vi "Read Language Selection UTF-16 LE.vi"(8 "error in (no error)":errorcluster, 11 "LanguageSelection file":path) -> (0 "error out":errorcluster, 3 "Language Selection":T1)   [LabVIEW 2019, in "Language Selection.lvlib"]
doc: "Convert translation from JSON format.\n- - -\nCopyright (c) 2026, Merecs Engineering GmbH"
uses:
  Language Selection.lvlib
  TypeDefs/Cluster Language Configuration.ctl
  Cluster Settings Data.ctl
  TypeDefs/Cluster Language.ctl
  TypeDefs/Cluster PropertyTranslation.ctl
  TypeDefs/Enum Property Type.ctl
  7aaee674-9885-4f51-b860-93eee7d62f3f.vi
  private/Hex-String To String.vi
  <vilib>/addons/Tools/Unicode/_subVIs/Convert ASCII to UTF-16LE (Scalar).vi
  <vilib>/addons/Tools/Unicode/_subVIs/Convert UTF-16LE to ASCII (Scalar).vi
  <vilib>/JDP Science/JSONtext/JSON text to Variant.vi
  <vilib>/JDP Science/JSONtext/LVClass Serializer/JSONtext LVClass Serializer.lvclass
  <vilib>/addons/Tools/Unicode/UI Unicode Tools.lvlib
panel:
  # "Connector Pane"
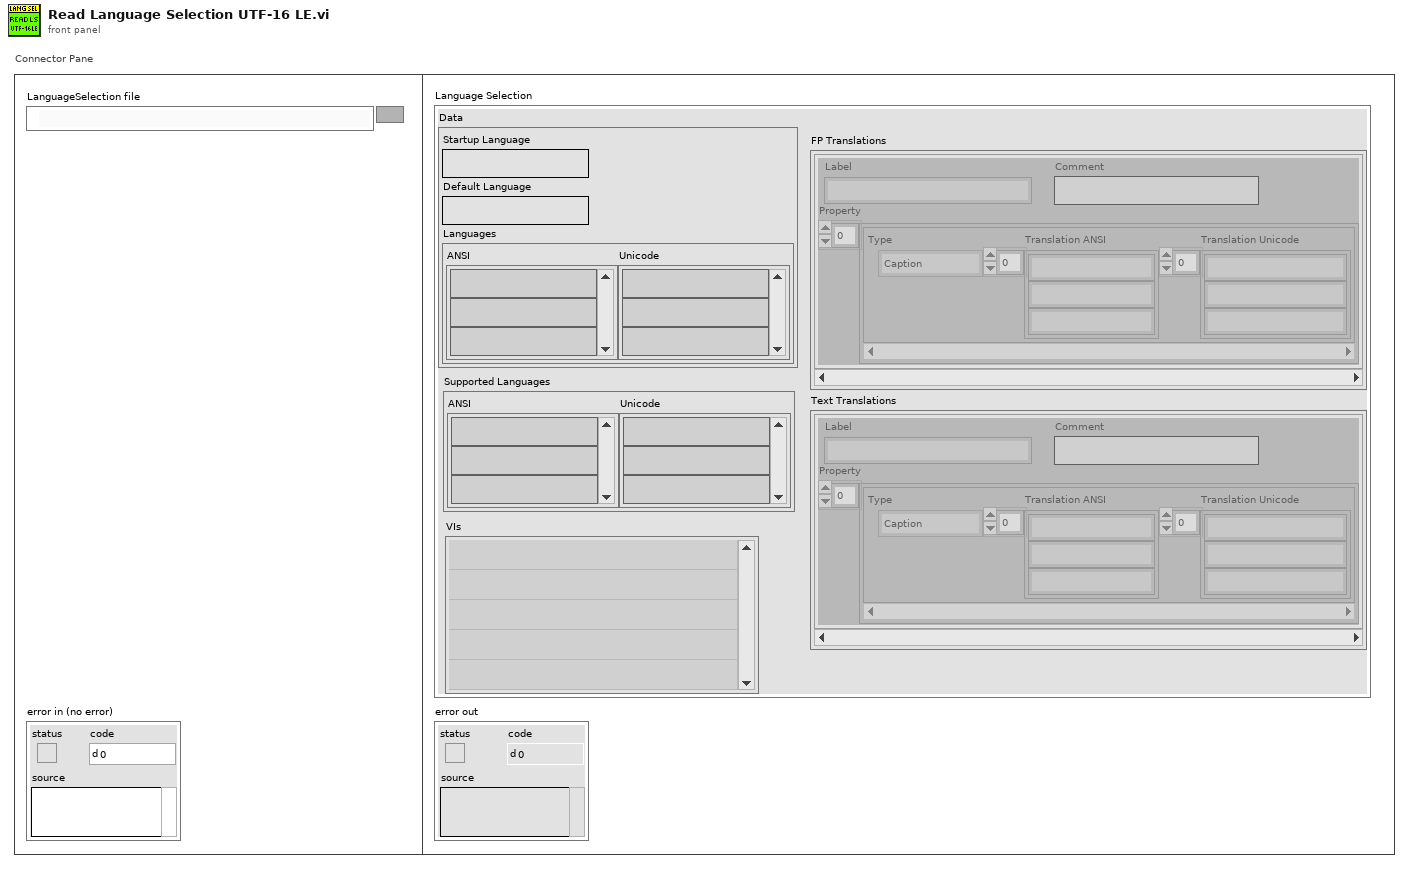
[diagram p1: front panel]
types:
  T1 = typedef "Language Selection.lvlib/Cluster Language Configuration.ctl" = cluster{"Data":T2, "Supported Languages":cluster{"ANSI":string[], "Unicode":string[]}, "VIs":path[], "FP Translations":T3[], "Text Translations":T3[]}
  T2 = typedef "Language Selection.lvlib/Cluster Settings Data.ctl" = cluster{"Startup Language":string, "Default Language":string, "Languages":cluster{"ANSI":string[], "Unicode":string[]}}
  T3 = typedef "Language Selection.lvlib/Cluster Language.ctl" = cluster{"Label":string, "Comment":string, "Property":T4[]}
  T4 = typedef "Language Selection.lvlib/Cluster PropertyTranslation.ctl" = cluster{"Type":T5, "Translation ANSI":string[], "Translation Unicode":string[]}
  T5 = typedef "Language Selection.lvlib/Enum Property Type.ctl" = enum16{"NA", "Caption", "String Value", "Boolean Text", "Ring Strings", "1D Array Elements", "2D Array Elements", "(MC)Listbox Header", "(MC)Listbox Items", "Tab Pages Names", "X & Y GraphChart", "Plot Names", "Table Headers", "Table Items", "TipStrip", "Combobox Strings", "Cursor Name", "Tree Col Headers"}
  T6 = enum16{"open", "replace", "create", "open or create", "replace or create", "replace or create with confirmation"}
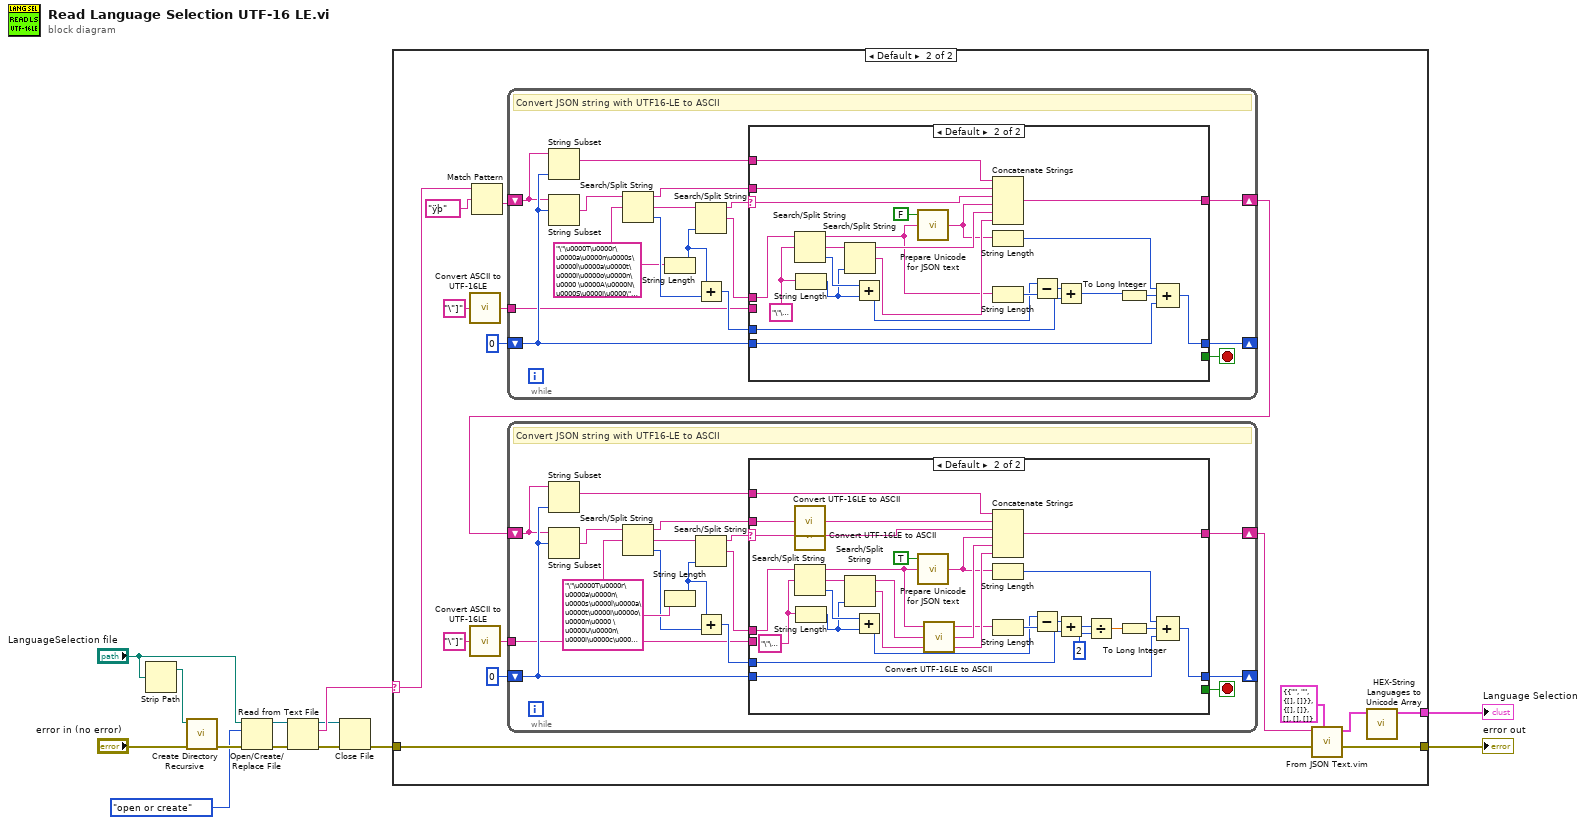
[diagram p0: block diagram]
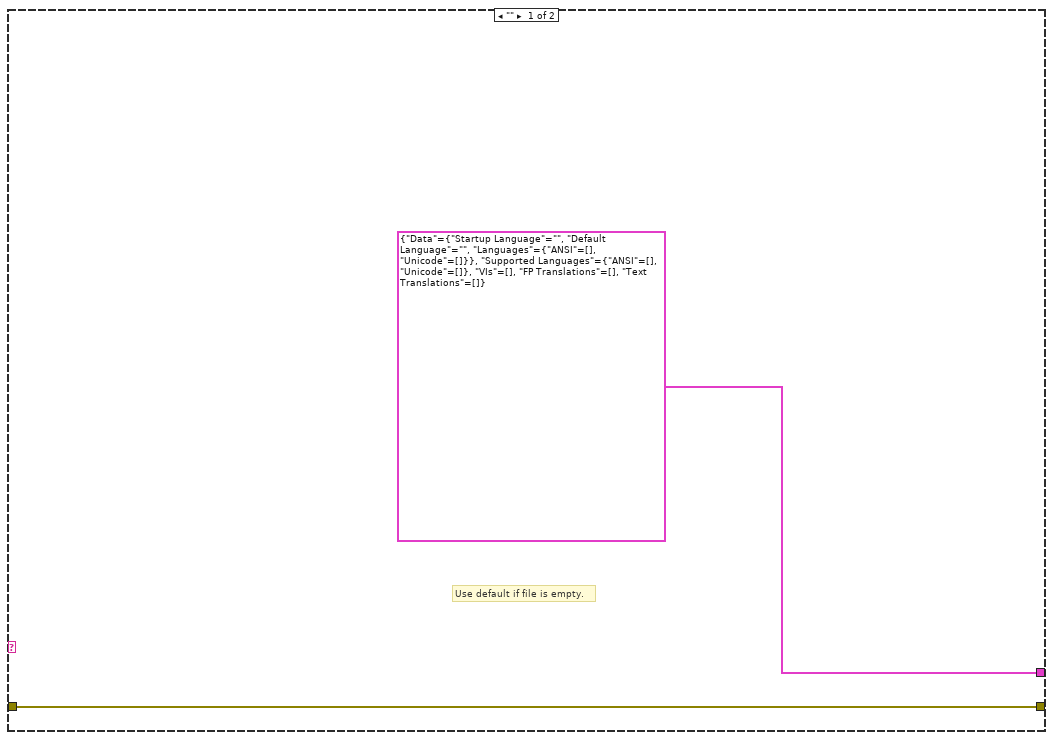
[diagram p2: hidden frame]
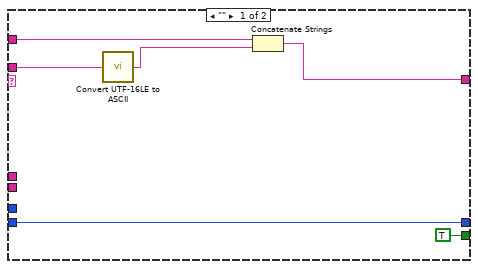
[diagram p3: hidden frame]
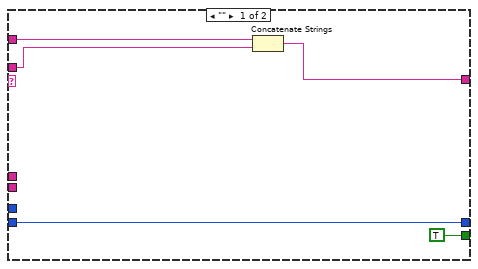
[diagram p4: hidden frame]
diagram:
  n1 = Strip Path(path="LanguageSelection file") -> (stripped path=w9:path)  [unwired: 1 out]
  n2 = call <vilib>:"Create Directory Recursive.vi"("error in (no error)"="error in (no error)", "directory"=w9) -> ("error out"=w7:errorcluster)  [unwired: 3 in, 2 out]
  n3 = Open/Create/Replace File(file path (use dialog)="LanguageSelection file", error in=w7, operation (0:open)=T6."open or create") -> (refnum out=w3:refnum<file>, error out=w4:errorcluster)  [unwired: 3 in, 1 out]
  n4 = Read from Text File(file (use dialog)=w3, error in=w4) -> (refnum out=w1:refnum<file>, text=w10:string, error out=w13:errorcluster)  [unwired: 2 in, 1 out]
  n5 = Close File(refnum=w1, error in=w13) -> (error out=w2:errorcluster)  [unwired: 1 out]
  n6 = case shown="Default" w10 {
    selector: w10 -> [_ w17]
    tunnel: w2 -> [w15 w29]
    tunnel: [w15 w28] -> w12
    tunnel: [T1 {"Data"={"Startup Language"="", "Default Language"="", "Languages"={"ANSI"=[], "Unicode"=[]}}, "Supported Languages"={"ANSI"=[], "Unicode"=[]}, "VIs"=[], "FP Translations"=[], "Text Translations"=[]} ("Config out") w16] -> w11
    frame "" {
      # "Use default if file is empty."
    }
    frame Default {
      n7 = call-poly <vilib>:"Convert ASCII to UTF-16LE.vi"("ASCII"="\"]" ("regular expression")) -> ("Unicode"=w26:string)  [unwired: 4 in]
      n8 = call-poly <vilib>:"Convert ASCII to UTF-16LE.vi"("ASCII"="\"]" ("regular expression")) -> ("Unicode"=w21:string)  [unwired: 4 in]
      n9 = Match Pattern(string=w17, regular expression="ÿþ" ("string")) -> (after substring=w23:string)  [unwired: 1 in, 3 out]
      n10 = while {
        shift-right: [w83] -> w20
        shift-left: w23 -> [w94]
        shift-right: [w96] -> _
        shift-left: 0 -> [w95]
        tunnel: w26 -> [w84]
        stop <- w97 stop-if-true
        w82 = "\"\u0000T\u0000r\u0000a\u0000n\u0000s\u0000l\u0000a\u0000t\u0000i\u0000o\u0000n\u0000 \u0000A\u0000N\u0000S\u0000I\u0000\"\u0000:\u0000[\u0000\"\u0000" ("Unicode 2")
        # "Convert JSON string with UTF16-LE to ASCII"
        n11 = String Subset(string=w94, length (rest)=w95) -> (substring=w93:string)  [unwired: 1 in]
        n12 = String Subset(string=w94, offset (0)=w95) -> (substring=w92:string)  [unwired: 1 in]
        n13 = Search/Split String(string=w92, search string/char (-)=w82) -> (substring before match=w91:string, match + rest of string=w90:string, offset of match=w86:i32)  [unwired: 1 in]
        n14 = String Length(string=w82) -> (length=w87:i32)
        n15 = Search/Split String(string=w90, offset (0)=w87) -> (substring before match=w89:string, match + rest of string=w88:string)  [unwired: 1 in, 1 out]
        n16 = Add(x=w87, y=w86) -> (x+y=w85:i32)
        n17 = case shown="Default" w89 {
          selector: w89 -> [_ w117]
          tunnel: w88 -> [_ w115]
          tunnel: w91 -> [w98 w118]
          tunnel: [w99 w125] -> w83
          tunnel: [TRUE _] -> w97
          tunnel: [w101 w121] -> w96
          tunnel: w95 -> [w101 w119]
          tunnel: w85 -> [_ w124]
          tunnel: w93 -> [w100 w123]
          tunnel: w84 -> [_ _]
          frame "" {
            n18 = Concatenate Strings(w100, w98) -> (w99:string)
          }
          frame Default {
            w105 = "\"\u0000]\u0000" ("Unicode 3")
            n19 = Search/Split String(string=w115, search string/char (-)=w105) -> (substring before match=w107:string, match + rest of string=w114:string, offset of match=w111:i32)  [unwired: 1 in]
            n20 = String Length(string=w105) -> (length=w110:i32)
            n21 = Search/Split String(string=w114, offset (0)=w110) -> (substring before match=w113:string, match + rest of string=w112:string)  [unwired: 1 in, 1 out]
            n22 = Add(x=w111, y=w110) -> (x+y=w109:i32)
            n23 = call "Prepare Unicode for JSON text.vi"("String in"=w107, "Unicode (True)"=FALSE) -> ("String out"=w106:string)  [unwired: 3 in]
            n24 = Concatenate Strings(w123, w118, w117, w106, w113, w112) -> (w125:string)
            n25 = String Length(string=w106) -> (length=w116:i32)
            n26 = String Length(string=w107) -> (length=w120:i32)
            n27 = Subtract(x=w109, y=w120) -> (x-y=w122:i32)
            n28 = Add(x=w122, y=w124) -> (x+y=w103:i32)
            n29 = To Long Integer(number=w103) -> (32bit integer=w108:i32)
            n30 = Compound Arithmetic op=ADD(w116, w108, w119) -> (w121:i32)
          }
        }
      }
      n31 = while {
        shift-right: [w43] -> w19
        shift-left: w20 -> [w44]
        shift-right: [w46] -> _
        shift-left: 0 -> [w45]
        tunnel: w21 -> [w32]
        stop <- w47 stop-if-true
        w39 = "\"\u0000T\u0000r\u0000a\u0000n\u0000s\u0000l\u0000a\u0000t\u0000i\u0000o\u0000n\u0000 \u0000U\u0000n\u0000i\u0000c\u0000o\u0000d\u0000e\u0000\"\u0000:\u0000[\u0000\"\u0000" ("regular expression")
        # "Convert JSON string with UTF16-LE to ASCII"
        n32 = String Subset(string=w44, length (rest)=w45) -> (substring=w42:string)  [unwired: 1 in]
        n33 = String Subset(string=w44, offset (0)=w45) -> (substring=w41:string)  [unwired: 1 in]
        n34 = Search/Split String(string=w41, search string/char (-)=w39) -> (substring before match=w40:string, match + rest of string=w38:string, offset of match=w34:i32)  [unwired: 1 in]
        n35 = String Length(string=w39) -> (length=w35:i32)
        n36 = Search/Split String(string=w38, offset (0)=w35) -> (substring before match=w37:string, match + rest of string=w36:string)  [unwired: 1 in, 1 out]
        n37 = Add(x=w35, y=w34) -> (x+y=w33:i32)
        n38 = case shown="Default" w37 {
          selector: w37 -> [_ w72]
          tunnel: w36 -> [_ w65]
          tunnel: w40 -> [w49 w74]
          tunnel: [w50 w81] -> w43
          tunnel: [TRUE _] -> w47
          tunnel: [w52 w77] -> w46
          tunnel: w45 -> [w52 w75]
          tunnel: w33 -> [_ w80]
          tunnel: w42 -> [w51 w79]
          tunnel: w32 -> [_ _]
          frame "" {
            n39 = call-poly <vilib>:"Convert UTF-16LE to ASCII.vi"("Unicode"=w49) -> ("ASCII"=w48:string)  [unwired: 4 in]
            n40 = Concatenate Strings(w51, w48) -> (w50:string)
          }
          frame Default {
            w55 = "\"\u0000]\u0000" ("Unicode 3")
            n41 = call-poly <vilib>:"Convert UTF-16LE to ASCII.vi"("Unicode"=w74) -> ("ASCII"=w73:string)  [unwired: 4 in]
            n42 = call-poly <vilib>:"Convert UTF-16LE to ASCII.vi"("Unicode"=w72) -> ("ASCII"=w71:string)  [unwired: 4 in]
            n43 = Search/Split String(string=w65, search string/char (-)=w55) -> (substring before match=w57:string, match + rest of string=w64:string, offset of match=w61:i32)  [unwired: 1 in]
            n44 = String Length(string=w55) -> (length=w60:i32)
            n45 = Search/Split String(string=w64, offset (0)=w60) -> (substring before match=w63:string, match + rest of string=w62:string)  [unwired: 1 in, 1 out]
            n46 = Add(x=w61, y=w60) -> (x+y=w59:i32)
            n47 = call "Prepare Unicode for JSON text.vi"("String in"=w57, "Unicode (True)"=TRUE) -> ("String out"=w56:string)  [unwired: 3 in]
            n48 = call-poly <vilib>:"Convert UTF-16LE to ASCII.vi"("Unicode"=w63) -> ("ASCII"=w70:string)  [unwired: 4 in]
            n49 = Concatenate Strings(w79, w73, w71, w56, w70, w62) -> (w81:string)
            n50 = String Length(string=w56) -> (length=w69:i32)
            n51 = String Length(string=w57) -> (length=w76:i32)
            n52 = Subtract(x=w59, y=w76) -> (x-y=w78:i32)
            n53 = Add(x=w78, y=w80) -> (x+y=w68:i32)
            n54 = Divide(x=w68, y=2) -> (x/y=w66:dbl)
            n55 = To Long Integer(number=w66) -> (32bit integer=w58:i32)
            n56 = Compound Arithmetic op=ADD(w69, w58, w75) -> (w77:i32)
          }
        }
      }
      n57 = call "From JSON Text.vim"("Data Type and Default Value"=T1 {"Data"={"Startup Language"="", "Default Language"="", "Languages"={"ANSI"=[], "Unicode"=[]}}, "Supported Languages"={"ANSI"=[], "Unicode"=[]}, "VIs"=[], "FP Translations"=[], "Text Translations"=[]} ("Config Data out"), "error in (no error)"=w29, "JSON"=w19) -> ("error out"=w28:errorcluster, "Data out"=w27:T1)  [unwired: 7 in]
      n58 = call "HEX-String Languages to Unicode Array.vi"("Config in"=w27) -> ("Config out"=w16:T1)  [unwired: 10 in]
    }
  }
  "error out" <- w12
  "Language Selection" <- w11
